vi "CSM - Resolve Node Module.vi"(10 "Node Name":string) -> (2 "CSM Module Name":string)   [LabVIEW 2017, in "Communicable State Machine.lvlib"]
doc: "Parses the corresponding CSM module name from an Advanced Mode node name.\n\nFor example:\n- For a Worker Mode node named `module#59703F3AD837`, the result is `module`.\n- For a Chain of Responsibility Mode node named `module$1`, the result is `module`.\n\n-- <b>Controls</b> --\n- <b>CSM Module Name</b>: CSM module name.\n- <b>Node Name</b>: Node name."
uses:
  Communicable State Machine.lvlib
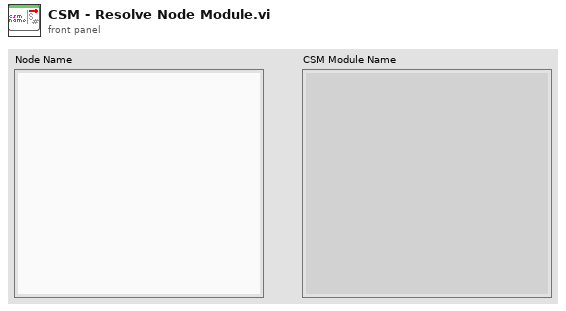
[diagram p1: front panel]
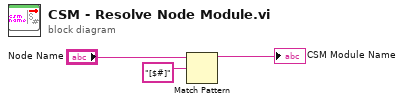
[diagram p0: block diagram]
diagram:
  n1 = Match Pattern(string="Node Name", regular expression="[$#]") -> (before substring=→"CSM Module Name":string)  [unwired: 1 in, 3 out]
